vi "TCP Server Launch Connection Process.vi"(8 "error out":errorcluster, 10 "Connection Data":T1, 11 "TCP Server RefNum":refnum<class "JKI TCP Server.lvclass">) -> (0 "error":errorcluster)   [LabVIEW 2020, in "JKI TCP Server.lvclass"]
uses:
  JKI TCP Server.lvclass
  _Data Structures/TCP Server Connection Process Data Cluster.ctl
  _Processes/TCP Server Connection Process.vi
  JKI TCP Server.lvclass/JKI TCP Server.ctl
panel:
  # "Copyright © 2004-2008 JKI. All rights reserved.\n\nAuthor: Jim Kring [jim.kring@jameskring.com]\n\nThis library is provided \"AS IS\" ,WITHOUT WARRANTIES OR \nCONDITIONS OF ANY KIND, either express or implied.\n\nJames Kring, Inc. -- http://www.jameskring.com"
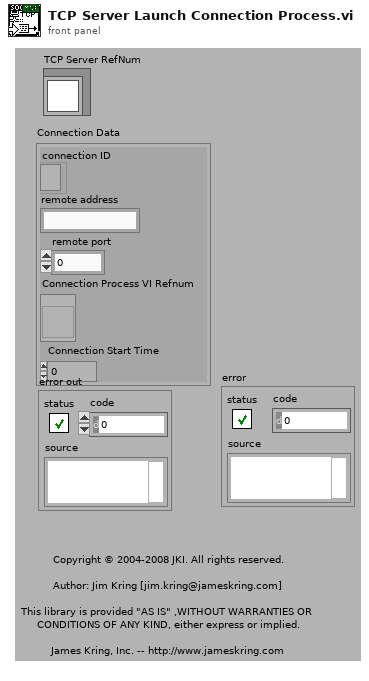
[diagram p1: front panel]
types:
  T1 = typedef "JKI TCP Server.lvclass/TCP Server Connection Process Data Cluster.ctl" = cluster{"connection ID":refnum<k5>, "remote address":string, "remote port":u16, "Connection Process VI Refnum":refnum<vi>, "Connection Start Time":u32}
  T2 = typedef "JKI TCP Server.lvclass/TCP Server Connection Info Cluster.ctl" = cluster{"connection ID":refnum<k5>, "Remote Address":string, "remote port":u16, "connection start time":u32}
  T3 = typedef "JKI TCP Server.lvclass/TCP Server Handler RefNum.ctl" = refnum<vi>
  T4 = cluster{"Connection Process VI Refnum":refnum<vi>, "TCP Handler VI RefNum":T3}
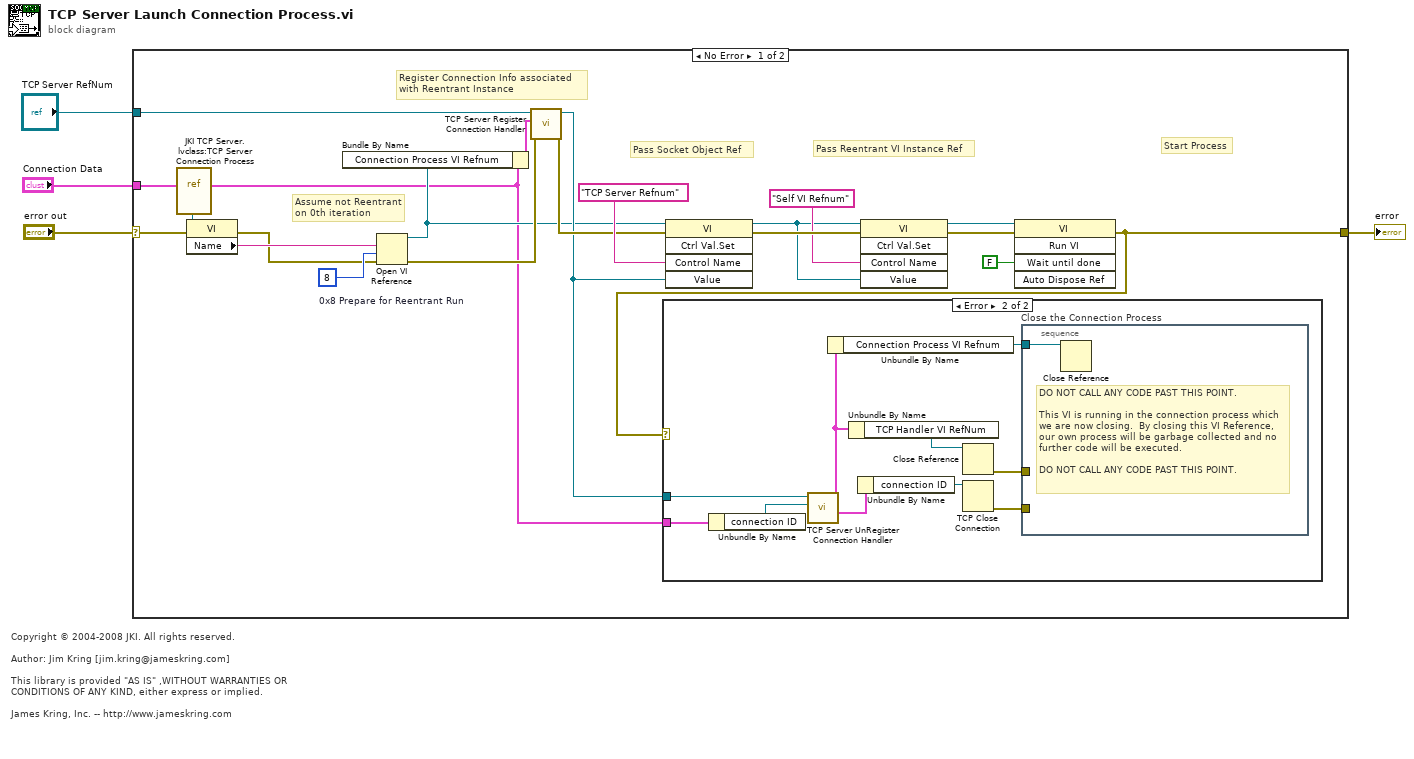
[diagram p0: block diagram]
diagram:
  # "Copyright © 2004-2008 JKI. All rights reserved.\n\nAuthor: Jim Kring [jim.kring@jameskring.com]\n\nThis library is provided \"AS IS\" ,WITHOUT WARRANTIES OR \nCONDITIONS OF ANY KIND, either express or implied.\n\nJames Kring, Inc. -- http://www.jameskring.com"
  n1 = case shown="No Error" "error out" {
    selector: "error out" -> [w6 w36]
    tunnel: "Connection Data" -> [w12 _]
    tunnel: "TCP Server RefNum" -> [w24 _]
    tunnel: [w11 w36] -> w2
    frame No Error {
      w21 = 8  # 0x8 Prepare for Reentrant Run
      # "Register Connection Info associated with Reentrant Instance"
      # "Pass Socket Object Ref"
      # "Pass Reentrant VI Instance Ref"
      # "Assume not Reentrant on 0th iteration"
      # "Start Process"
      n2 = vi-ref "JKI TCP Server.lvclass:TCP Server Connection Process.vi"() -> (w8:refnum<vi>)
      n3 = property class="VI"(reference=w8, error in=w6) -> (error out=w5:errorcluster, "Name"=w7:string)  [unwired: 1 out]
      n4 = Open VI Reference(vi path=w7, options=w21, error in (no error)=w5) -> (vi reference=w13:refnum<vi>, error out=w19:errorcluster)  [unwired: 3 in]
      n5 = Bundle By Name(cluster=w12, "Connection Process VI Refnum"=w13) -> (w20:T1)
      n6 = call "TCP Server Register Connection Handler.vi"("error in (no error)"=w19, "Connection Data"=w20, "RefNum"=w24) -> ("error out"=w18:errorcluster, "dup RefNum"=w14:refnum<class "JKI TCP Server.lvclass">)  [unwired: 6 in, 1 out]
      n7 = invoke class="VI" method="Ctrl Val.Set"(reference=w13, error in=w18, "Control Name"="TCP Server Refnum", "Value"=w14) -> (reference out=w15:refnum<vi>, error out=w17:errorcluster)  [unwired: 1 in, 3 out]
      n8 = invoke class="VI" method="Ctrl Val.Set"(reference=w15, error in=w17, "Control Name"="Self VI Refnum", "Value"=w15) -> (reference out=w10:refnum<vi>, error out=w9:errorcluster)  [unwired: 1 in, 3 out]
      n9 = invoke class="VI" method="Run VI"(reference=w10, error in=w9, "Wait until done"=FALSE) -> (error out=w11:errorcluster)  [unwired: 2 in, 4 out]
      n10 = case shown="Error" w11 {
        tunnel: w14 -> [_ w27]
        tunnel: w12 -> [_ w26]
        frame No Error {
        }
        frame Error {
          n11 = Unbundle By Name(w26) -> ("connection ID"=w25:refnum<k5>)
          n12 = call "TCP Server UnRegister Connection Handler.vi"("connection ID"=w25, "TCP Server RefNum"=w27) -> ("Connection Info"=w34:T2, "VI References"=w29:T4)  [unwired: 7 in, 1 out]
          n13 = Unbundle By Name(w29) -> ("Connection Process VI Refnum"=w30:refnum<vi>)
          n14 = Unbundle By Name(w29) -> ("TCP Handler VI RefNum"=w28:T3)
          n15 = Unbundle By Name(w34) -> ("connection ID"=w33:refnum<k5>)
          n16 = Close Reference(reference=w28) -> (error out=w31:errorcluster)  [unwired: 1 in]
          n17 = TCP Close Connection(connection ID=w33) -> (error out=w32:errorcluster)  [unwired: 2 in, 1 out]
          n18 = stacked-sequence "Close the Connection Process" {
            tunnel: w30 -> [w35]
            tunnel: w32 -> [_]
            tunnel: w31 -> [_]
            frame #0 {
              # "DO NOT CALL ANY CODE PAST THIS POINT.\n\nThis VI is running in the connection process which we are now closing.  By closing this VI Reference, our own process will be garbage collected and no further code will be executed.\n\nDO NOT CALL ANY CODE PAST THIS POINT."
              n19 = Close Reference(reference=w35) -> ()  [unwired: 1 in, 1 out]
            }
          }
        }
      }
    }
    frame Error {
    }
  }
  "error" <- w2
